vi "ziModGetUnsignedIntegerData.vi"(8 "Error In":errorcluster, 10 "ModResults":T2, 11 "ModHandle In":T5 {"ModHandle" format="0x%08x"; "Conn" format="0x%08x"}) -> (0 "Error Out":errorcluster, 2 "ModIUnsignedntegerData":T1[](array[typedef]), 3 "ModHandle Out":T5 {"ModHandle" format="0x%08x"; "Conn" format="0x%08x"}, 4 "Value":u64[](array[numeric]))   [LabVIEW 2009, in "Zurich Instruments LabOne.lvlib"]
doc: "Use this vi to get IntegerData from a ModResult returned from ziModGetNextNode.vi. It return an array of IntegerData."
uses:
  <instrlib>/Zurich Instruments LabOne/Zurich Instruments LabOne.lvlib
  <instrlib>/Zurich Instruments LabOne/Public/Modules/ziTypeModHandle.ctl
  <instrlib>/Zurich Instruments LabOne/Public/Modules/ziTypeModResults.ctl
  <instrlib>/Zurich Instruments LabOne/Public/Data/ziTypePollType.ctl
  <instrlib>/Zurich Instruments LabOne/Public/Modules/ziTypeModGenericHeader.ctl
  <instrlib>/Zurich Instruments LabOne/Public/Data/ziTypeUnsignedIntegerData.ctl
  <instrlib>/Zurich Instruments LabOne/Public/Data/ziTypeIntegerDataTSGrid.ctl
  <instrlib>/Zurich Instruments LabOne/Private/ziLV32.dll
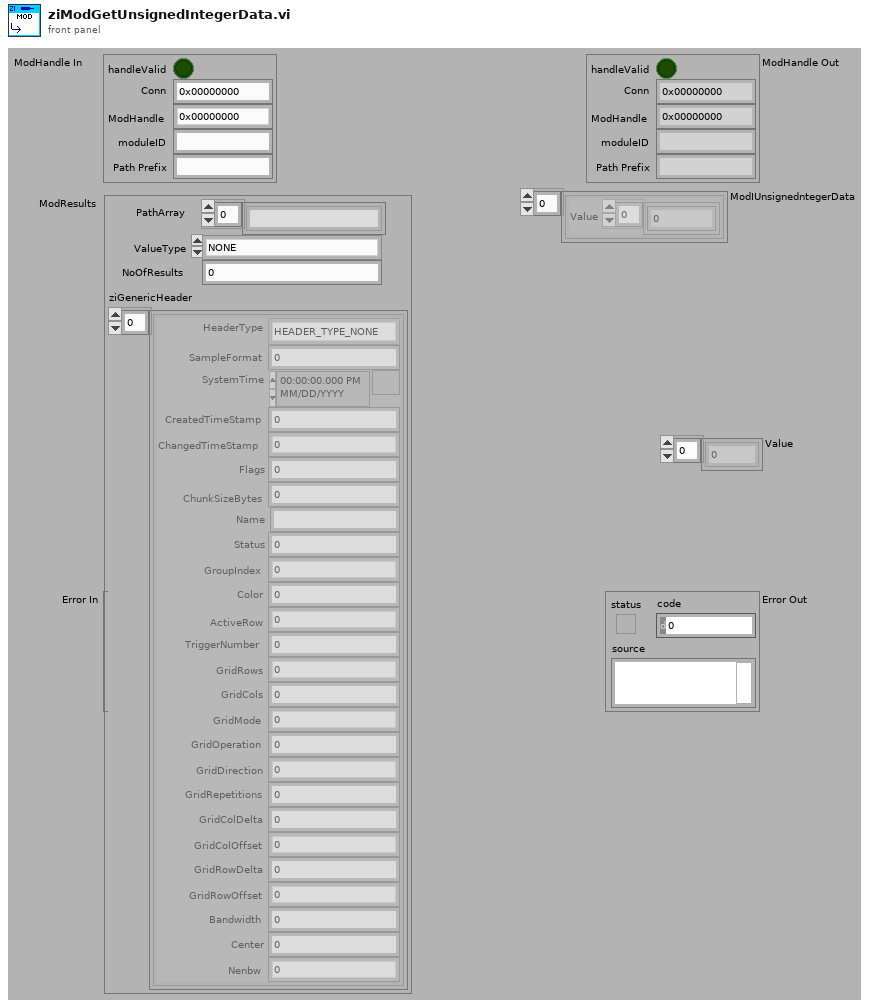
[diagram p1: front panel]
types:
  T1 = typedef "Zurich Instruments LabOne.lvlib/ziTypeUnsignedIntegerData.ctl" = cluster{"Value":u64[]}
  T2 = typedef "Zurich Instruments LabOne.lvlib/ziTypeModResults.ctl" = cluster{"PathArray":string[], "ValueType":T3, "NoOfResults":u64, "ziGenericHeader":T4[]}
  T3 = typedef "Zurich Instruments LabOne.lvlib/ziTypePollType.ctl" = enum16{"NONE", "DOUBLE_DATA", "INTEGER_DATA", "DEMOD_SAMPLE", "SCOPE_WAVE_HF2", "AUXIN_SAMPLE", "DIO_SAMPLE", "BYTE_ARRAY", "PWA_WAVE", "9", "10", "11", "12", "13", "14", "15", "TREE_CHANGE_DEPRI", "17", "ERROR", "19", "20", "21", "22", "23", "24", "25", "26", "27", "28", "29", "30", "31", "DOUBLE_DATA_TS", "INTEGER_DATA_TS", "34", "SCOPE_WAVE", "SCOPE_WAVE_EX", "37", "BYTE_ARRAY_TS", "39", "40", "41", "42", "43", "44", "45", "CNT_DATA", "47", "TREE_CHANGE", "49", "50", "51", "52", "53", "54", "55", "56", "57", "58", "59", "60", "61", "62", "63", "SWEEPER_DATA", "SPECTRUM_DATA", "ADVISOR_DATA", "VECTOR_DATA", "IMP_DATA", "SHF_GENERATOR_WAVEFORM_DATA", "SHF_RESULT_LOGGER_DATA", "SHF_SCOPE_DATA", "DEMOD_VECTOR", "73", "PID_VECTOR", "UNSIGNED_INTEGER_DATA"}
  T4 = typedef "Zurich Instruments LabOne.lvlib/ziTypeModGenericHeader.ctl" = cluster{"HeaderType":enum8{"HEADER_TYPE_NONE", "HEADER_TYPE_SWTRIGGER", "HEADER_TYPE_SWEEPER"}, "SampleFormat":u8, "SystemTime":timestamp, "CreatedTimeStamp":u64, "ChangedTimeStamp":u64, "Flags":u32, "ChunkSizeBytes":u64, "Name":string, "Status":u32, "GroupIndex":u32, "Color":u32, "ActiveRow":u32, "TriggerNumber":u64, "GridRows":u32, "GridCols":u32, "GridMode":u32, "GridOperation":u32, "GridDirection":u32, "GridRepetitions":u32, "GridColDelta":dbl, "GridColOffset":dbl, "GridRowDelta":dbl, "GridRowOffset":dbl, "Bandwidth":dbl, "Center":dbl, "Nenbw":dbl}
  T5 = typedef "Zurich Instruments LabOne.lvlib/ziTypeModHandle.ctl" = cluster{"handleValid":bool, "Conn":u64, "ModHandle":u64, "moduleID":string, "Path Prefix":string}
  T6 = typedef "Zurich Instruments LabOne.lvlib/ziTypeIntegerDataTSGrid.ctl" = cluster{"Timestamp (ticks)":u64[][], "Value":i64[][]}
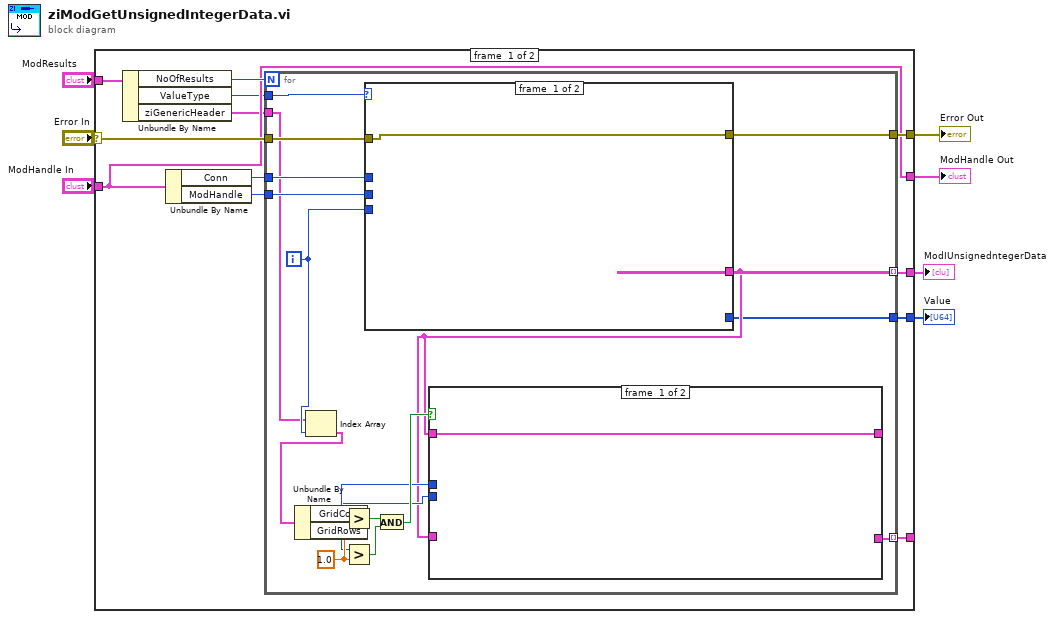
[diagram p0: block diagram]
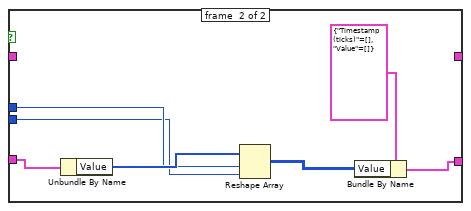
[diagram p2: hidden frame]
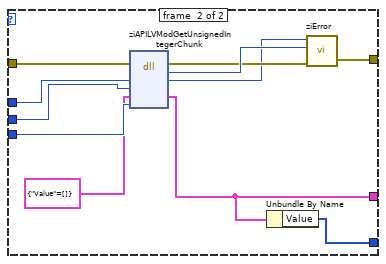
[diagram p3: hidden frame]
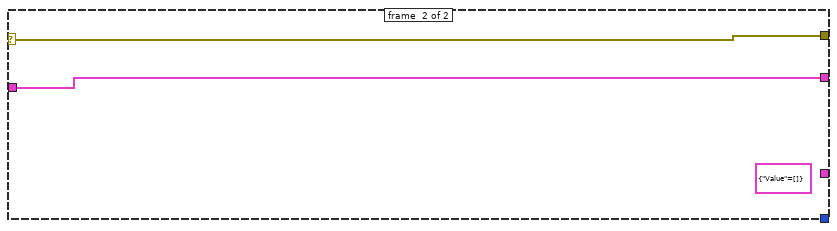
[diagram p4: hidden frame]
diagram:
  n1 = case shown="No Error" "Error In" {
    selector: "Error In" -> [w14 w57]
    tunnel: [w15 w57] -> w3
    tunnel: [w13 w58] -> w6
    tunnel: "ModHandle In" -> [w13 w58]
    tunnel: "ModResults" -> [w17 _]
    tunnel: [w12 _] -> w2
    tunnel: [w9 _] -> _
    tunnel: [w8 _] -> w1
    frame #0 {
      n2 = Unbundle By Name(w17) -> ("NoOfResults"=w16:u64, "ValueType"=w11:T3, "ziGenericHeader"=w10:T4[])
      n3 = Unbundle By Name(w13) -> ("Conn"=w19:u64, "ModHandle"=w18:u64)
      n4 = for {
        N: w16 -> [_]
        tunnel: w19 -> [w36]
        tunnel: w18 -> [w35]
        tunnel: [w34] -> w15
        tunnel: w14 -> [w33]
        tunnel: [w25] -> w12 mode=indexing
        tunnel: w11 -> [w32]
        tunnel: w10 -> [w21]
        tunnel: [w24] -> w9 mode=indexing
        tunnel: [w20] -> w8
        i -> [w22]
        w31 = 1.0 ("y")
        n5 = Index Array(array=w21, index=w22) -> (element=w23:T4)
        n6 = Unbundle By Name(w23) -> ("GridCols"=w26:u32, "GridRows"=w27:u32)
        n7 = Greater?(x=w26, y=w31) -> (0:w29:bool)
        n8 = Greater?(x=w27, y=w31) -> (0:w30:bool)
        n9 = case shown="\"UNSIGNED_INTEGER_DATA\"" w32 {
          tunnel: w36 -> [_ w56]
          tunnel: w35 -> [_ w55]
          tunnel: w22 -> [_ w54]
          tunnel: [w45 w53] -> w34
          tunnel: w33 -> [w45 w50]
          tunnel: [_ w47] -> w25
          tunnel: [_ w46] -> w20
          frame #0 {
          }
          frame #1 {
            n10 = dll-call lib="C:/Program Files (x86)/National Instruments/LabVIEW 2009/instr.lib/Zurich Instruments LabOne/Private/ziLV*.*" fn="ziAPILVModGetUnsignedIntegerChunk"(error in=w50, "Conn"=w56, "ModHandle"=w55, "UnsignedIntegerData"=T1 {"Value"=[]} ("IntegerSample 3"), "chunk_idx"=w54) -> (error out=w51:errorcluster, "return type"=w52:u32, "Conn"=w49:u64, "UnsignedIntegerData"=w47:T1)  [unwired: 4 in, 1 out]
            n11 = Unbundle By Name(w47) -> ("Value"=w46:u64[])
            n12 = call <instrlib>:"ziError.vi"("Conn"=w49, "ziErrorCode"=w52, "Error In"=w51) -> ("Error Out"=w53:errorcluster)  [unwired: 2 in, 1 out]
          }
        }
        n13 = And(x=w29, y=w30) -> (x .and. y?=w28:bool)
        n14 = case shown="True" w28 {
          tunnel: w25 -> [_ w44]
          tunnel: w25 -> [w37 _]
          tunnel: [w37 _] -> _
          tunnel: w27 -> [_ w42]
          tunnel: w26 -> [_ w40]
          tunnel: [_ w41] -> w24
          frame #0 {
          }
          frame #1 {
            n15 = Unbundle By Name(w44) -> ("Value"=w43:u64[])
            n16 = Reshape Array(w43, w42, w40) -> (w39:u64[][])
            n17 = Bundle By Name(cluster=T6 {"Timestamp (ticks)"=[], "Value"=[]} ("IntegerData"), "Value"=w39) -> (w41:T6)
          }
        }
      }
    }
    frame #1 {
      (unwired) T1 {"Value"=[]} ("IntegerSample 2")
    }
  }
  "Error Out" <- w3
  "ModHandle Out" <- w6
  "ModIUnsignedntegerData" <- w2
  "Value" <- w1
